vi "Close.vi"(8 "error in (no error)":errorcluster, 11 "Data in":refnum<class "CTI_GPIO_DigitalOut.lvclass">) -> (0 "error out":errorcluster, 3 "Data out":refnum<class "CTI_GPIO_DigitalOut.lvclass">)   [LabVIEW 2021, in "CTI_GPIO_DigitalOut.lvclass"]
doc: "Abstract Data Classes 2.1.1.13\nTim Streeter - TSA\nCopyright (c) 2025, TSA"
uses:
  CTI_GPIO_DigitalOut.lvclass
  CTI_GPIO_DigitalOut.lvclass/CTI_GPIO_DigitalOut.ctl
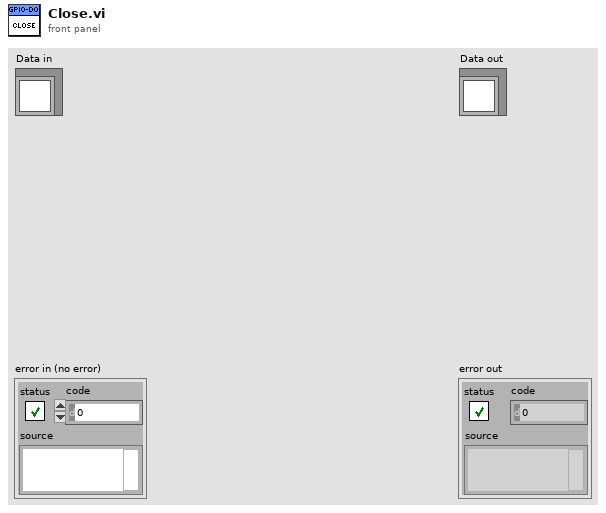
[diagram p1: front panel]
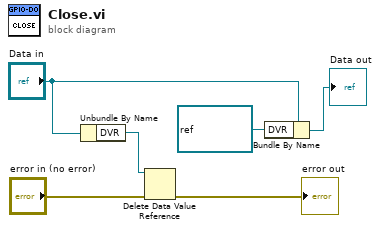
[diagram p0: block diagram]
diagram:
  n1 = Unbundle By Name("Data in") -> ("DVR"=w4:refnum<data-value>)
  n2 = Delete Data Value Reference(data value reference=w4, error in="error in (no error)") -> (error out=→"error out":errorcluster)  [unwired: 1 out]
  n3 = Bundle By Name(cluster="Data in", "DVR"=refnum<data-value> refnum) -> (→"Data out":refnum<class "CTI_GPIO_DigitalOut.lvclass">)
